vi "AprilTag_GetAll.vi"(11 "AprilTag":T5={"ID"=0, "POSE3D"={"Translation3d"={"X"=0.0, "Y"=0.0, "Z"=0.0}, "Rotation3d"={"Q_quaternion"={"R"=1.0, "V"=[0.0, 0.0, 0.0]}}}} {"POSE3D"."Translation3d"."Z" format="%14.3f"; "POSE3D"."Translation3d"."Y" format="%14.3f"; "POSE3D"."Translation3d"."X" format="%14.3f"}) -> (1 "POSE3D":T1={"Translation3d"={"X"=0.0, "Y"=0.0, "Z"=0.0}, "Rotation3d"={"Q_quaternion"={"R"=1.0, "V"=[0.0, 0.0, 0.0]}}} {"Translation3d"."Z" format="%14.3f"; "Translation3d"."Y" format="%14.3f"; "Translation3d"."X" format="%14.3f"}, 3 "ID":i32)   [LabVIEW 2019, in "Trajectory_Library.lvlib"]
doc: "Get individual items from the AprilTag data cluster\n\nInputs:\n -- AprilTag -- AprilTag -- Data cluster storing AprilTag\n\nOutputs:\n -- ID -- Integer -- AprilTag ID value\n -- POSE3d -- Pose3d -- Position of the April Tag. This could be relative or absolute. It is most often absolute position."
uses:
  Trajectory_Library.lvlib
  TypeDef/AprilTag.ctl
  TypeDef/POSE3D.ctl
  TypeDef/TRANSLATION3D.ctl
  TypeDef/ROTATION3D.ctl
  TypeDef/QUATERNION.ctl
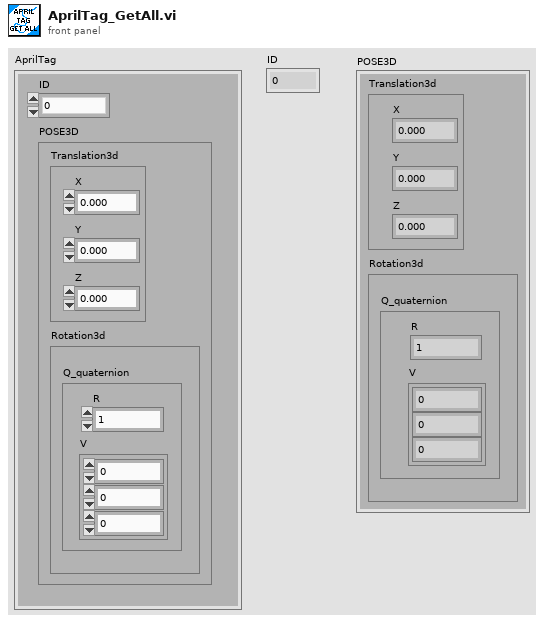
[diagram p1: front panel]
types:
  T1 = typedef "Trajectory_Library.lvlib/POSE3D.ctl" = cluster{"Translation3d":T2, "Rotation3d":T3}
  T2 = typedef "Trajectory_Library.lvlib/TRANSLATION3D.ctl" = cluster{"X":dbl, "Y":dbl, "Z":dbl}
  T3 = typedef "Trajectory_Library.lvlib/ROTATION3D.ctl" = cluster{"Q_quaternion":T4}
  T4 = typedef "Trajectory_Library.lvlib/QUATERNION.ctl" = cluster{"R":dbl, "V":dbl[]}
  T5 = typedef "Trajectory_Library.lvlib/AprilTag.ctl" = cluster{"ID":i32, "POSE3D":T1}
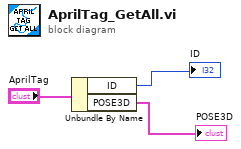
[diagram p0: block diagram]
diagram:
  n1 = Unbundle By Name("AprilTag") -> ("ID"=→"ID":i32, "POSE3D"=→"POSE3D":T1)
